vi "Test - Read Text Without CR.vi"(8 "error in (no error)":errorcluster, 11 "File":path) -> (0 "error out":errorcluster, 3 "Text":string)   [LabVIEW 2024]
doc: "Reads a whole text file and removes every carriage return, so files written with CR LF and files written with LF compare equal.\n\nGenerated by: Claude"
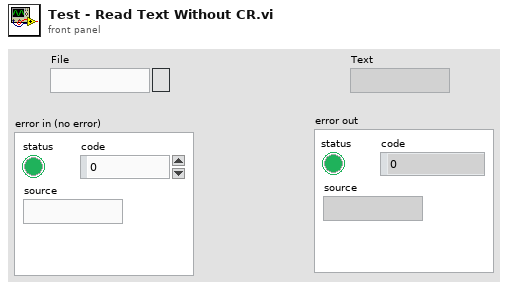
[diagram p1: front panel]
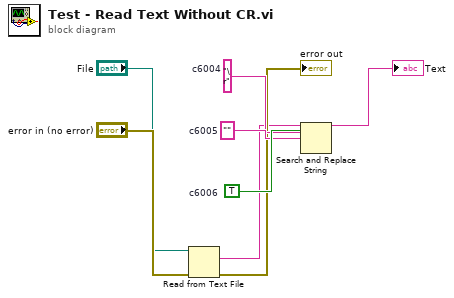
[diagram p0: block diagram]
diagram:
  w7 = TRUE  # c6006
  w6 = ""  # c6005
  w5 = "\r"  # c6004
  n1 = Read from Text File(file (use dialog)="File", error in="error in (no error)") -> (text=w3:string, error out=→"error out":errorcluster)  [unwired: 2 in, 2 out]
  n2 = Search and Replace String(replace all?=w7, input string=w3, search string=w5, replace string=w6) -> (result string=→"Text":string)  [unwired: 4 in, 3 out]
